vi "VIH Constant - ProjFile - Root Tag Attributes.vi"() -> (3 "Root Tag Attributes":cluster{"Name":string, "Value":string}[](array[cluster]))   [LabVIEW 2014]
doc: "::: VI Helpeks :::\nCopyright (c) 2000-2026 Konstantin Shifershteyn. All rights reserved."
panel:
  # "VI Helpeks\nCopyright (c) 2012-2026 Konstantin Shifershteyn"
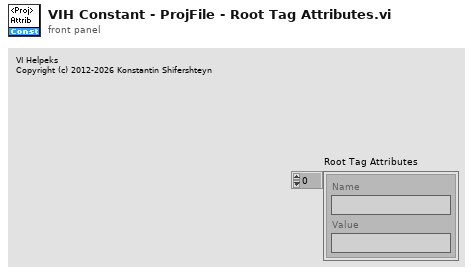
[diagram p1: front panel]
types:
  T1 = cluster{"Name":string, "Product Version":string}[]
  T2 = cluster{"Product Name":string, "Short Name":string, "Product Version":string, "Release Timestamp":string, "Developer":string, "Copyright":string}
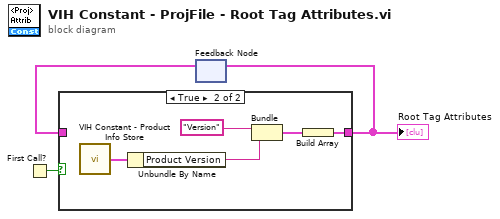
[diagram p0: block diagram]
diagram:
  n1 = First Call?() -> (First Call?: T/F=w3:bool)
  n2 = feedback #1() -> (w1:T1)  [unwired: 1 in]
  n3 = case shown="True" w3 {
    tunnel: [w4 w5] -> w2
    tunnel: w1 -> [w4 _]
    frame False {
    }
    frame True {
      n4 = call "VIH Constant - Product Info Store.vi"() -> ("Product Info"=w9:T2)
      n5 = Unbundle By Name(w9) -> ("Product Version"=w7:string)
      n6 = Bundle("Name"="Version", "Product Version"=w7) -> (w6:cluster{"Name":string, "Product Version":string})  [unwired: 1 in]
      n7 = Build Array(w6) -> (w5:T1)
    }
  }
  "Root Tag Attributes" <- w2
  n8 = feedback-in #1(w2) -> ()
